vi "RemoteVI Remote Hooks.vi"(0 "panel?":bool, 1 "mods":u8, 2 "VI name":string, 3 "origin":cluster{"x":i32, "y":i32}, 5 "tips in":string="tips []", 6 "splitters in":string="splitters []", 7 "bars in":T1(array[cluster]), 11 "error in":errorcluster) -> (4 "tips out":string, 8 "splitters out":string, 9 "bars out":T1(array[cluster]), 15 "error out":errorcluster)   [LabVIEW 2020, in "RemoteVI Hooks.lvlib"]
doc: "Runs INSIDE another LabVIEW process (a LabVIEW-built application or another LabVIEW) whose window RemoteVI shares over VI Server (docs\\architecture.md, Window targets, VI Server route). RemoteVI Server opens this VI in that application instance by its path on disk (Open VI Reference with the application reference), sets its controls (Set Control Value), runs it (Run VI, wait until done) and reads its indicators - so the work below happens in the target's own process and UI thread, exactly as for a panel of RemoteVI's own LabVIEW. panel? FALSE: mods is written into the key state of the target's UI thread (RemoteVI Set Modifier Keys.vi, SetKeyboardState in the UI thread - the only way Shift, Ctrl and Alt reach LabVIEW, which reads them with GetKeyState). panel? TRUE: the VI called VI name is opened in this process and its tip strips and splitter bars are read (RemoteVI Read Tips.vi, RemoteVI Read Splitters.vi) with origin; tips out, splitters out and bars out are the messages (tips in, splitters in and bars in on an error). Not a member of RemoteVI.lvlib on purpose: an application built with RemoteVI holds the library's VIs without front panels, and a VI without a front panel cannot take Set Control Value; this VI is always loaded from disk with its panel and calls the library VIs as subVIs (those the target already holds, or loaded from source next to this file)."
uses:
  RemoteVI Hooks.lvlib
  source/RemoteVI.lvlib
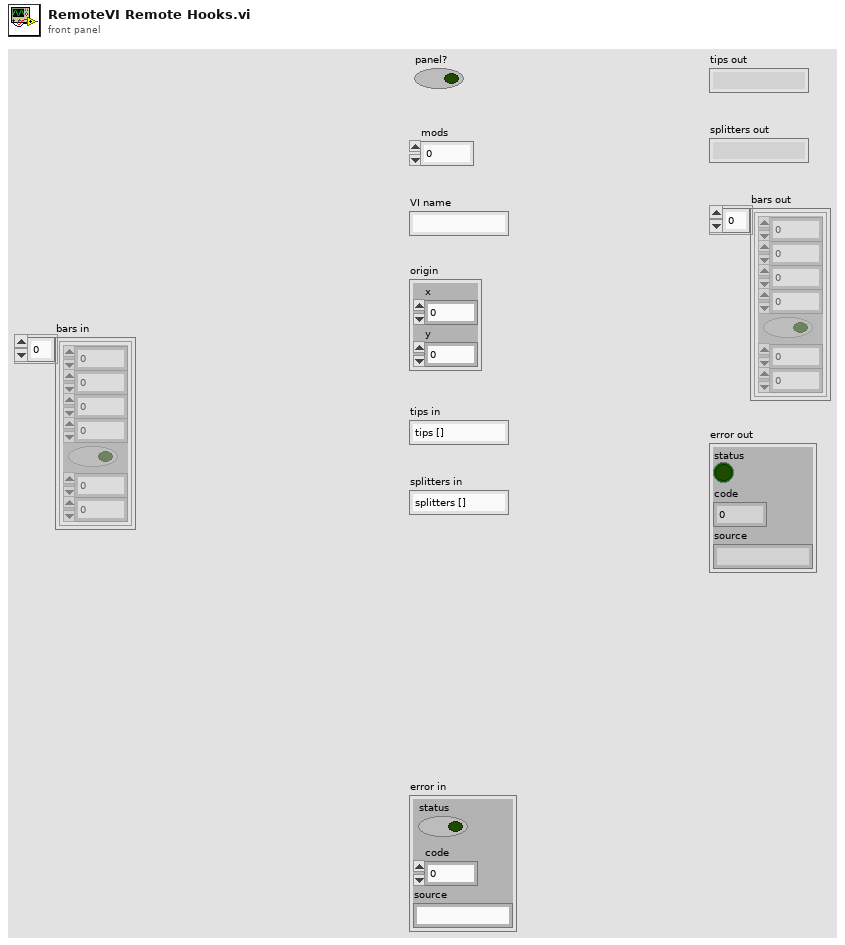
[diagram p1: front panel]
types:
  T1 = cluster{"x":i32, "y":i32, "w":i32, "h":i32, "vertical":bool, "min":i32, "max":i32}[]
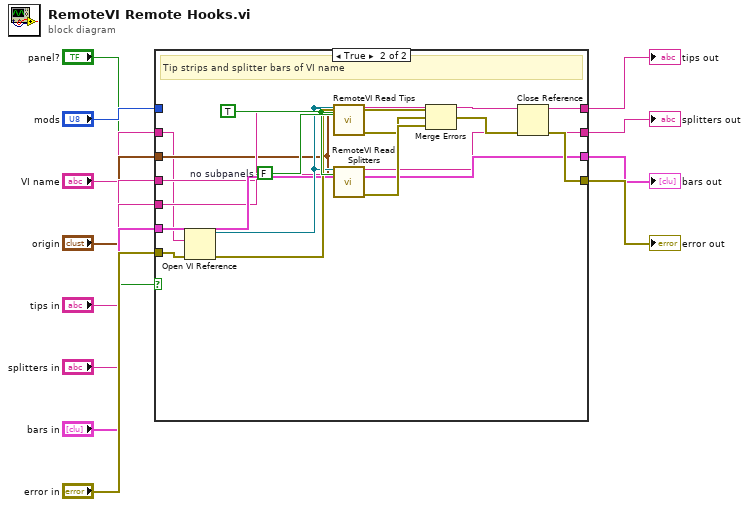
[diagram p0: block diagram]
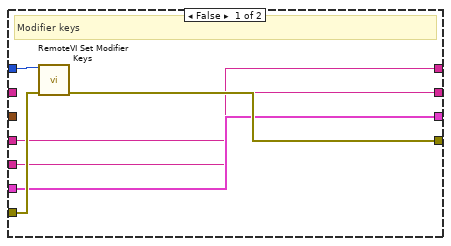
[diagram p2: hidden frame]
diagram:
  n1 = case shown="True" "panel?" {
    tunnel: "mods" -> [w13 _]
    tunnel: "VI name" -> [_ w19]
    tunnel: "origin" -> [_ w20]
    tunnel: "tips in" -> [w14 w21]
    tunnel: "splitters in" -> [w15 w22]
    tunnel: "bars in" -> [w16 w23]
    tunnel: "error in" -> [w17 w24]
    tunnel: [w14 w29] -> w9
    tunnel: [w15 w31] -> w10
    tunnel: [w16 w32] -> w11
    tunnel: [w18 w35] -> w12
    frame False {
      # "Modifier keys"
      n2 = call "RemoteVI Set Modifier Keys.vi"("mods"=w13, "error in"=w17) -> ("error out"=w18:errorcluster)  [unwired: 13 in]
    }
    frame True {
      w28 = FALSE  # no subpanels
      w27 = TRUE
      # "Tip strips and splitter bars of VI name"
      n3 = Open VI Reference(vi path=w19, error in (no error)=w24) -> (vi reference=w25:refnum<vi>, error out=w26:errorcluster)  [unwired: 4 in]
      n4 = call "RemoteVI Read Tips.vi"("VI"=w25, "refresh?"=w27, "origin"=w20, "message in"=w21, "subpanels?"=w28) -> ("message out"=w29:string, "error out"=w30:errorcluster)  [unwired: 9 in]
      n5 = call "RemoteVI Read Splitters.vi"("VI"=w25, "refresh?"=w27, "origin"=w20, "message in"=w22, "bars in"=w23) -> ("message out"=w31:string, "bars out"=w32:T1, "error out"=w33:errorcluster)  [unwired: 8 in]
      n6 = Merge Errors(w26, w30, w33) -> (w34:errorcluster)
      n7 = Close Reference(reference=w25, error in (no error)=w34) -> (error out=w35:errorcluster)
    }
  }
  "tips out" <- w9
  "splitters out" <- w10
  "bars out" <- w11
  "error out" <- w12
